vi "Write String Direct.vi"(8 "error in (no error)":errorcluster, 10 "Data":string, 11 "CIFTag in":refnum<class "CIF_Iceoryx_Chn_String.lvclass">) -> (0 "error out":errorcluster, 3 "CIFTag out":refnum<class "CIF_Iceoryx_Chn_String.lvclass">)   [LabVIEW 2021, in "CIF_Iceoryx_Chn_String.lvclass"]
uses:
  CIF_Iceoryx_Chn_String.lvclass
  CIFChannels/CIFChannels.lvclass/CIFChannels.ctl
  CIF_Iceoryx_Chn_String.lvclass/CIF_Iceoryx_Chn_String.ctl
  CIF_Iceoryx_BB/CIF_Iceoryx_BB.lvclass/CIF_Iceoryx_BB.ctl
  ChannelCommon/typedef/Errors.ctl
  46c631c6-c319-459f-b22a-b0c63d4769f6.vi
  CIFChannels/Accessors/Read Tag Forced.vi
  <vilib>/CIF Foundation/CIF Iceoryx/SubVIs/Get Path.vi
  <vilib>/CIF Foundation/CIF Iceoryx/SubVIs/Convert Error.vi
  <vilib>/CIF Foundation/CIF Iceoryx/Refnum/BB Writer from Refnum.vi
  <vilib>/CIF Foundation/CIF Iceoryx/SubVIs/Convert Error Core.vi
  ChannelCommon/Utilities/Add Error Core.vi
  ChannelCommon/ChannelCommon.lvlib
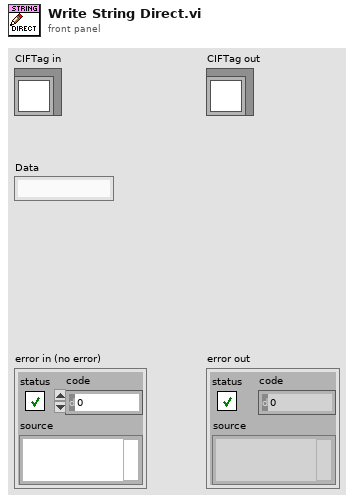
[diagram p1: front panel]
types:
  T1 = typedef "Iceoryx.lvlib/BB Writer Refnum.ctl" = cluster{"refnum":u64, "BB Writer":enum8{"bb_writer"}}
  T2 = typedef "ChannelCommon.lvlib/Errors.ctl" = enum8{"gRPC Server Not Found", "Duplicate Channel", "Missing Channel", "Incorrect Type", "Flatten Error", "Unflatten Data", "Channel Length", "Plugin Connection", "gRPC Server Connection", "FIFO Unflatten", "Required Override", "Remove Not Found", "Multi Sub Not Supported", "Primary Already Connected", "Backpressure Not Supported", "Unable to Increase Buffer", "Data too Large"}
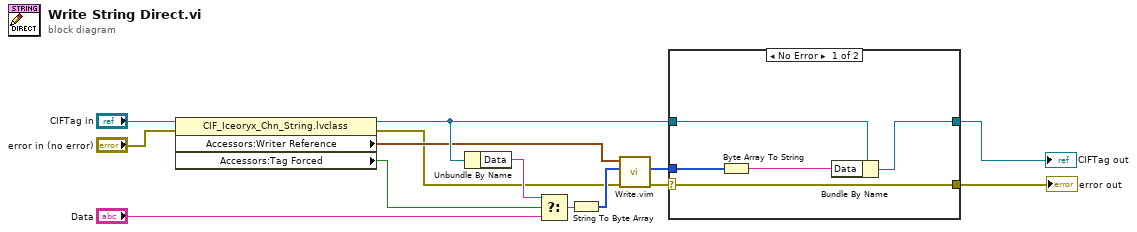
[diagram p0: block diagram]
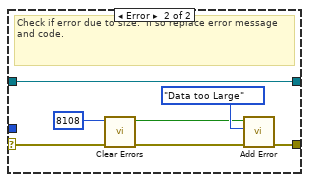
[diagram p2: hidden frame]
diagram:
  n1 = property class="CIF_Iceoryx_Chn_String.lvclass"(reference="CIFTag in", error in="error in (no error)") -> (reference out=w3:refnum<class "CIF_Iceoryx_Chn_String.lvclass">, error out=w1:errorcluster, "Accessors:Writer Reference"=w2:T1, "Accessors:Tag Forced"=w4:bool)
  n2 = Unbundle By Name(w3) -> ("Data"=w9:string)
  n3 = Select(t=w9, s=w4, f="Data") -> (s? t:f=w8:string)
  n4 = String To Byte Array(string=w8) -> (unsigned byte array=w6:u8[])
  n5 = call "Write.vim"("error in (no error)"=w1, "Data In"=w6, "Writer Reference"=w2) -> ("error out"=w5:errorcluster, "Data Out"=w7:u8[])  [unwired: 7 in]
  n6 = case shown="No Error" w5 {
    selector: w5 -> [w15 w22]
    tunnel: w3 -> [w19 w26]
    tunnel: [w18 w26] -> w11
    tunnel: w7 -> [w17 _]
    tunnel: [w15 w24] -> w10
    frame No Error {
      n7 = Byte Array To String(unsigned byte array=w17) -> (string=w16:string)
      n8 = Bundle By Name(cluster=w19, "Data"=w16) -> (w18:refnum<class "CIF_Iceoryx_Chn_String.lvclass">)
    }
    frame Error {
      # "Check if error due to size.  If so replace error message and code."
      n9 = call <vilib>:"Clear Errors.vi"("error in (no error)"=w22, "specific error code to clear (0: all)"=8108) -> ("error out"=w21:errorcluster, "specific error cleared?"=w20:bool)  [unwired: 4 in]
      n10 = call "Add Error.vi"("error in (no error)"=w21, "Error"=Errors."Data too Large", "Insert Error"=w20) -> ("error out"=w24:errorcluster)  [unwired: 8 in]
    }
  }
  "error out" <- w10
  "CIFTag out" <- w11
